vi "Moteur_Encodeur.vi"() -> ()   [LabVIEW 2017]
uses:
  <vilib>/Platform/TimedLoop/XDataNode/XDataNode.xnode
  <vilib>/Platform/TimedLoop/XDataNode/nitl_modes.ctl
  <vilib>/Platform/TimedLoop/XDataNode/XDNodeRunTimeDep.lvlib
  <vilib>/Platform/TimedLoop/XDataNode/wakeup.ctl
  <vilib>/Platform/TimedLoop/XDataNode/timing_clust.ctl
  <vilib>/myRIO/Common/Instrument Driver Framework/myRIO v1.0/Encoder/typedefs/Encoder Count Direction Enum.ctl
  <vilib>/myRIO/Common/Instrument Driver Framework/myRIO v1.0/Encoder/typedefs/Encoder Signal Mode.ctl
  <vilib>/myRIO/Common/Instrument Driver Framework/myRIO v1.0/Encoder/typedefs/Encoder Channels Enum.ctl
  <vilib>/myRIO/Common/Instrument Driver Framework/Utilities/typedefs/Generic FPGA Reference.ctl
  <vilib>/myRIO/Common/Instrument Driver Framework/Utilities/typedefs/myRIO v1.0 Reference.ctl
  <vilib>/myRIO/Common/Instrument Driver Framework/Utilities/typedefs/Hardware Version Enum.ctl
  <vilib>/myRIO/Common/Instrument Driver Framework/Utilities/typedefs/myRIO Generic Hardware Reference.ctl
  <vilib>/myRIO/Instrument Drivers/Onboard IO/Encoder/typedefs/Encoder Reference.ctl
  <vilib>/myRIO/Instrument Drivers/Onboard IO/Encoder/Encoder.lvlib
  <vilib>/myRIO/Instrument Drivers/Onboard IO/Encoder/vis/Read.vi
  <vilib>/myRIO/Common/Instrument Driver Framework/myRIO v1.0/Encoder/typedefs/Encoder Configuration v1.0.ctl
  <vilib>/userdefined/High Color/nirio_resource_hc.ctl
  <vilib>/myRIO/Common/Instrument Driver Framework/myRIO v1.0/Encoder/vis/myRIO v1.1 Open Encoder.vi
  <vilib>/myRIO/Common/Instrument Driver Framework/myRIO v1.0/Encoder/vis/myRIO v1.0 Configure Encoder.vi
  <vilib>/myRIO/Instrument Drivers/Onboard IO/Encoder/vis/myRIO Encoder Open.xnode
  <vilib>/myRIO/Common/Instrument Driver Framework/Utilities/vis/Is FPGA Ref Available.vi
  <vilib>/myRIO/Express VI/Onboard IO/Encoder/Encoder Express VI.xnode
panel:
  out "Graphe Delta d":dbl(graph)
  out "Graphe Delta Pulse":i32(graph)
  out "Graphe Duty D":dbl(graph)
  out "Duty Droit":dbl
  out "Duty Gauche":dbl
  in  "Duty ref":dbl=0.58
  out "Delta Pulse":i32
  out "Delta d":dbl
  out "Graphe Count 2":i32(graph)
  out "Graphe Count":i32(graph)
  in  "Pulse / tour":dbl=400.0
  out "distance cm  2":dbl
  out "angle  2":dbl
  out "tour  2":dbl
  out "Overflow?  2":bool
  out "Counter Direction 2":enum16{"Counting Up", "Counting Down"}(ring)
  out "Pulse 2":i32
  out "distance cm  3":dbl
  out "angle":dbl
  out "tour":dbl
  out "Overflow?":bool
  out "Counter Direction":enum16{"Counting Up", "Counting Down"}(ring)
  out "Pulse":i32
  in  "stop":bool
  # "A"
  # "B"
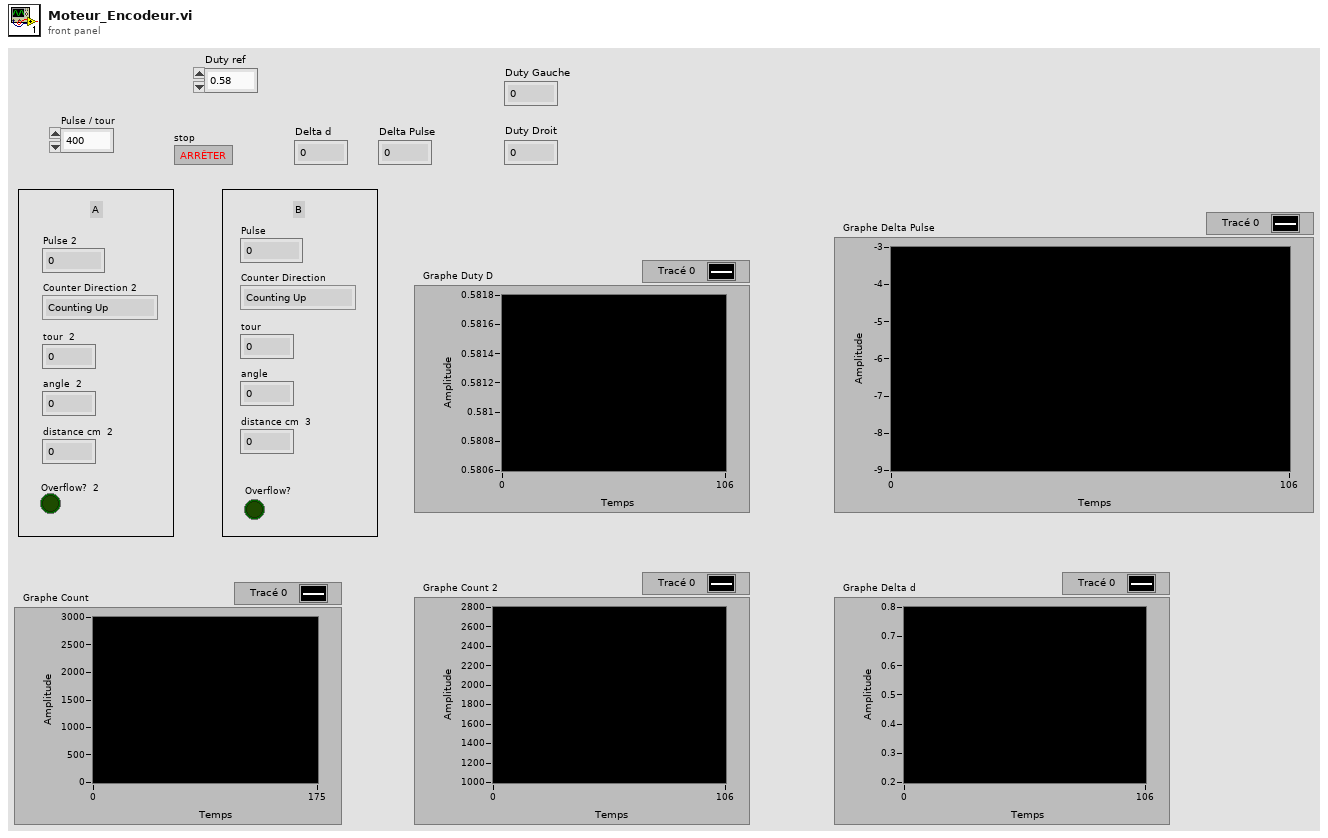
[diagram p1: front panel]
types:
  T1 = typedef "XDNodeRunTimeDep.lvlib/timing_clust.ctl" = cluster{"Expected End [f-1]":u64, "Actual End [f-1]":u64, "Finished Late? [f-1]":bool, "Expected End [i-1]":u64, "Actual End [i-1]":u64, "Finished Late? [i-1]":bool, "Expected Start [i]":u64, "Actual Start [i]":u64, "Expected Start [f]":u64, "Actual Start [f]":u64, "Source Name":string, "Structure Name":string, "Period":i64, "Deadline":i64, "Offset":i64, "Start":i64, "Priority":i32, "Timeout":i32, "Mode":T2, "Wakeup Reason":T3, "Error":errorcluster, "Source Type":string, "Secondary Source Type":string, "Global End Time":u64, "Global Start Time":u64, "Frame Duration":u64, "Iteration Duration":u64, "Assigned CPU":i32, "I/O Scan Engine Mode":u32}
  T2 = typedef "XDNodeRunTimeDep.lvlib/nitl_modes.ctl" = enum32{"No Change", "Process missed periods, maintain original phase", "Discard missed periods, maintain original phase", "Process missed periods, ignore original phase", "Discard missed periods, ignore original phase"}
  T3 = typedef "XDNodeRunTimeDep.lvlib/wakeup.ctl" = enum32{"Normal", "Aborted", "Asynchronous wakeup", "Timing source error", "Timed loop error", "Timeout"}
  T4 = typedef "Encoder.lvlib/Encoder Reference.ctl" = cluster{"myRIO Reference":T5, "Encoder Channels Enum":T9}
  T5 = typedef "myRIO Generic Hardware Reference.ctl" = cluster{"myRIO Model":T6, "myRIO Hardware Reference":T7}
  T6 = typedef "Hardware Version Enum.ctl" = enum16{"Unknown", "myRIO-1900", "myRIO-1950", "roboRIO", "NI ELVIS RIO CM"}
  T7 = typedef "myRIO v1.0 Reference.ctl" = cluster{"Generic FPGA Reference":T8, "Allow multiple opens":bool}
  T8 = typedef "Generic FPGA Reference.ctl" = refnum<k20>
  T9 = typedef "Encoder Channels Enum.ctl" = enum16{"Not Connected", "C/ENC0", "C/ENC1", "A/ENC", "B/ENC", "DIO/ENC0", "DIO/ENC1", "DIO/ENC2", "DIO/ENC3", "DIO/ENC4"}
  T10 = typedef "Encoder Signal Mode.ctl" = enum16{"Quadrature phase signal", "Step and direction signal"}
  T11 = typedef "nirio_resource_hc.ctl" = tag
  T12 = typedef "Encoder Count Direction Enum.ctl" = enum16{"Counting Up", "Counting Down"}
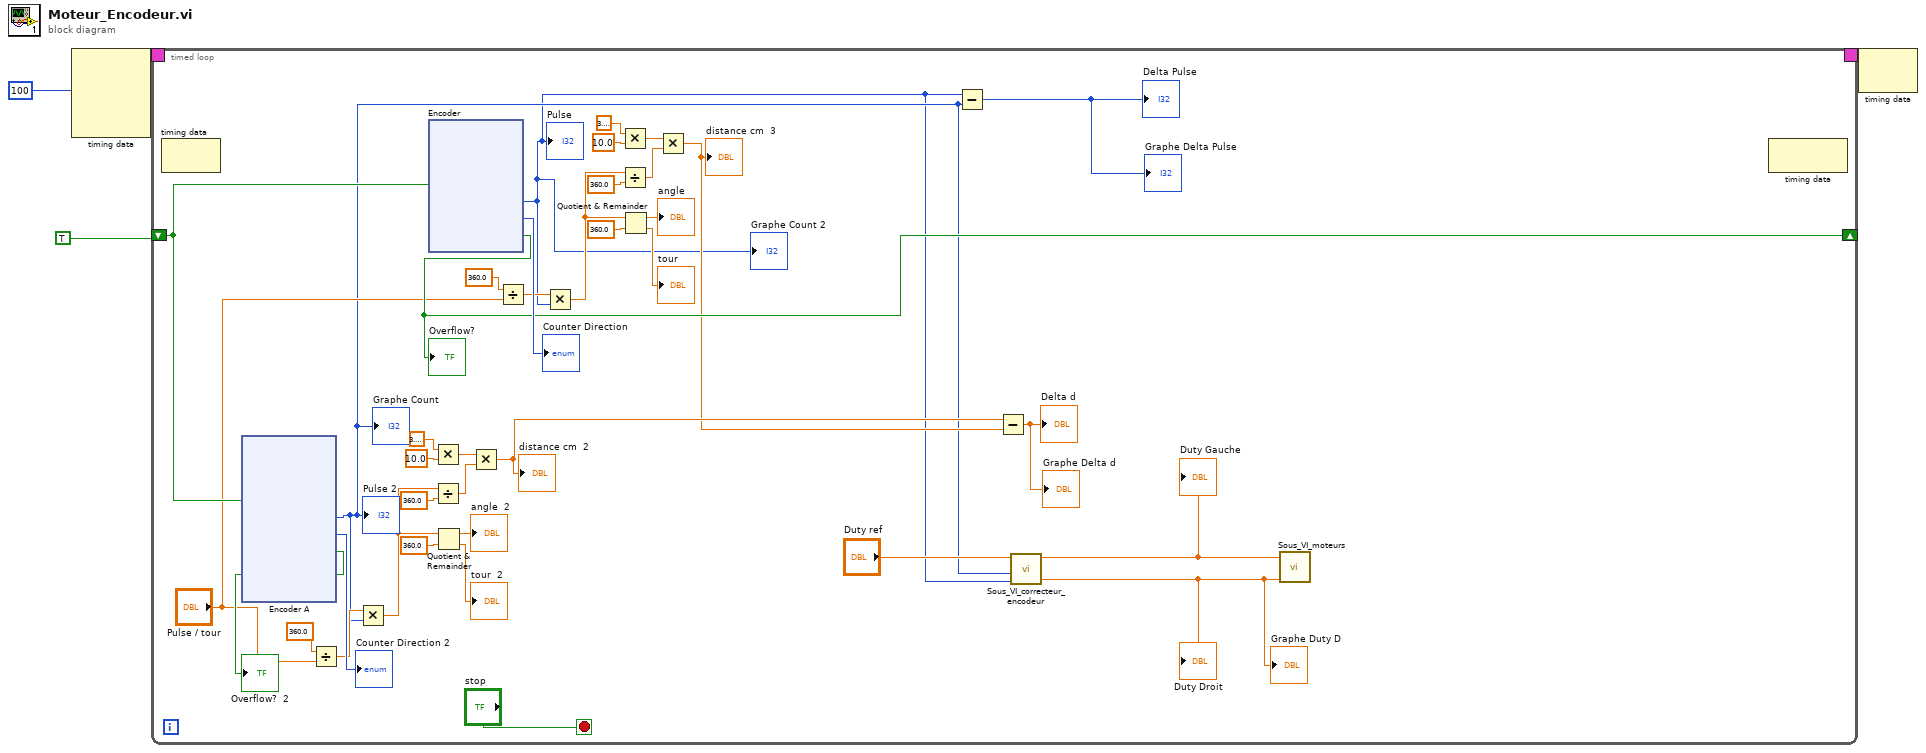
[diagram p0: block diagram]
diagram:
  n1 = node-c288(i64 100 ("Période")) -> (w4:T1)  [unwired: 3 in]
  n2 = timed-loop {
    timing: w4 -> [_]
    timing-out: [_] -> w3
    shift-right: [w16] -> _
    shift-left: TRUE -> [w17]
    stop <- "stop" stop-if-true
    n3 = node-c288() -> ()  [unwired: 1 in, 1 out]
    n4 = xnode "Encoder A"("Reset Counter"=w17) -> ("Counter Value"=w9:i32, "Counter Direction"=→"Counter Direction 2":T12, "Overflow?"=→"Overflow?  2":bool)  [unwired: 1 in, 1 out]
    "Pulse 2" <- w9
    "Graphe Count" <- w9
    n5 = Divide(x=360.0, y="Pulse / tour") -> (x/y=w19:dbl)
    n6 = Multiply(x=w19, y=w9) -> (x*y=w18:dbl)
    n7 = xnode "Encoder"("Reset Counter"=w17) -> ("Counter Value"=w8:i32, "Counter Direction"=→"Counter Direction":T12, "Overflow?"=w16:bool)  [unwired: 1 in, 1 out]
    "Pulse" <- w8
    "Overflow?" <- w16
    "Graphe Count 2" <- w8
    n8 = Multiply(x=3.141592653589793, y=10.0) -> (x*y=w24:dbl)
    n9 = Divide(x=w18, y=360.0) -> (x/y=w28:dbl)
    n10 = Quotient & Remainder(x=w18, y=360.0) -> (x-y*floor(x/y)=→"angle  2":dbl, floor(x/y)=→"tour  2":dbl)
    n11 = Multiply(x=w24, y=w28) -> (x*y=w13:dbl)
    "distance cm  2" <- w13
    n12 = Divide(x=360.0, y="Pulse / tour") -> (x/y=w31:dbl)
    n13 = Multiply(x=w31, y=w8) -> (x*y=w30:dbl)
    n14 = Multiply(x=3.141592653589793, y=10.0) -> (x*y=w36:dbl)
    n15 = Divide(x=w30, y=360.0) -> (x/y=w40:dbl)
    n16 = Quotient & Remainder(x=w30, y=360.0) -> (x-y*floor(x/y)=→"angle":dbl, floor(x/y)=→"tour":dbl)
    n17 = Multiply(x=w36, y=w40) -> (x*y=w12:dbl)
    "distance cm  3" <- w12
    n18 = Subtract(x=w8, y=w9) -> (x-y=→"Delta Pulse" →"Graphe Delta Pulse":i32)
    n19 = Subtract(x=w13, y=w12) -> (x-y=→"Delta d" →"Graphe Delta d":dbl)
    n20 = call "Sous_VI_correcteur_encodeur.vi"("Pulse Droit"=w8, "Pulse Gauche"=w9, "Duty ref"="Duty ref") -> ("Duty Droit"=w7:dbl, "Duty Gauche"=w10:dbl)  [unwired: 7 in]
    "Duty Gauche" <- w10
    "Duty Droit" <- w7
    "Graphe Duty D" <- w7
    n21 = call "Sous_VI_moteurs.vi"("error in (no error)"=w7, "Moteur Gauche"=w10) -> ()  [unwired: 9 in, 1 out]
    n22 = node-c288() -> ()  [unwired: 1 in, 1 out]
  }
  n23 = node-c288(w3) -> ()  [unwired: 1 out]
